vi "stream array to channel.vi"(9 "Values":dbl[](array[numeric]), 10 "Timestamps":timestamp[](array[timestamp]) format="%<%x %.3X>T", 11 "channel":refnum<class "Channel.lvclass">) -> (0 "error out":errorcluster)   [LabVIEW 2020, in "nominal core steps.lvlib"]
doc: "Stream an array of timestamps and values to the channel."
uses:
  nominal core steps.lvlib
  <vilib>/Nominal/Nominal IO Client/submodules/nominal-streaming-labview-ffi/lv_src/Channel/Channel.lvclass
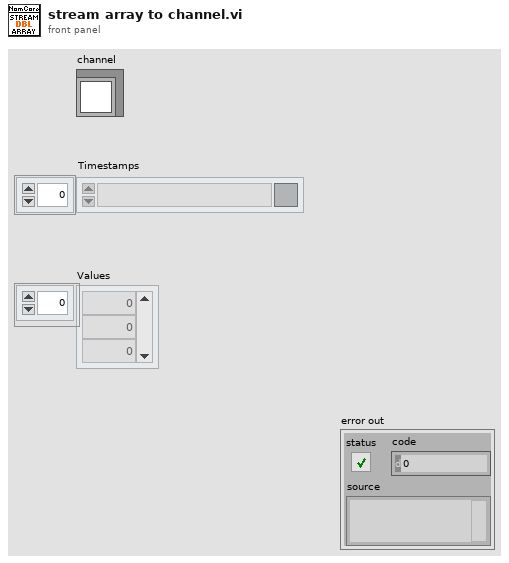
[diagram p1: front panel]
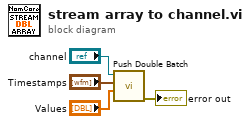
[diagram p0: block diagram]
diagram:
  n1 = call <vilib>:"Push Double Batch.vi"("Values"="Values", "Timestamps"="Timestamps", "Channel in"="channel") -> ("error out"=→"error out":errorcluster)  [unwired: 7 in, 1 out]
